vi "GLIMPSE Sequence Save.vi"(5 "Go? (F)":bool, 6 "Header file data":T2 {"Pixel depth" items=["8 bits", "16 bits", "Float", "Complex", "RGB", "HSL"]; "time of 1st frame, \nsec since 1/1/04" format="%.2f"}, 8 "Acquisition refnum array":refnum<file>[](array[refnum]), 9 "Black/White Levels":cluster{ext, ext}(slide)={1.0, 65535.0} scale=1.0..65535.0) -> ()   [LabVIEW 2015]
doc: "Saves a sequence either as a single movied file (SEQ, Stacked TIFF, or AVI) or as a directory full of individual frame images (Multiple TIFF). If more than one AOI is specified, each is saved in a separate, sequentially numbered file or directory. For stacked TIFF or AVI formats, also saves a separate .mat file with time information etc. See Save sequence file into movie.vi for information on the file format."
uses:
  Header file data.ctl
  Seq file v 1/Offset table.ctl
  Seq file v 1/Offset.ctl
  Seq file v 1/file number.ctl
  Header2 file data.ctl
  GLIMPSE Globals.vi
  AOI/AOI List Globals.vi
panel:
  out "Header2 file data 2":T1
  in  "Header2 file data":T1
  in  "AVI AOI Overlay\n(\"Entire Frames\" only)":bool
  in  "AVI Frames Per Second":u32=30
  out "Keep acquisition files open at end":bool=TRUE
  in  "Change File":bool
  out "Current movie directory":path=path "d:/1.glimpse"
  in  "AOI Options":i32(listbox)=1
  in  "stop":bool
  in  "Description Info (SEQ and stacked TIFF formats)":string
  in  "To":u32
  in  "From":u32
  in  "Frame Range Options":i32(listbox)
  in  "File Format Options":i32(listbox)
  # "Make any changes required, then press"
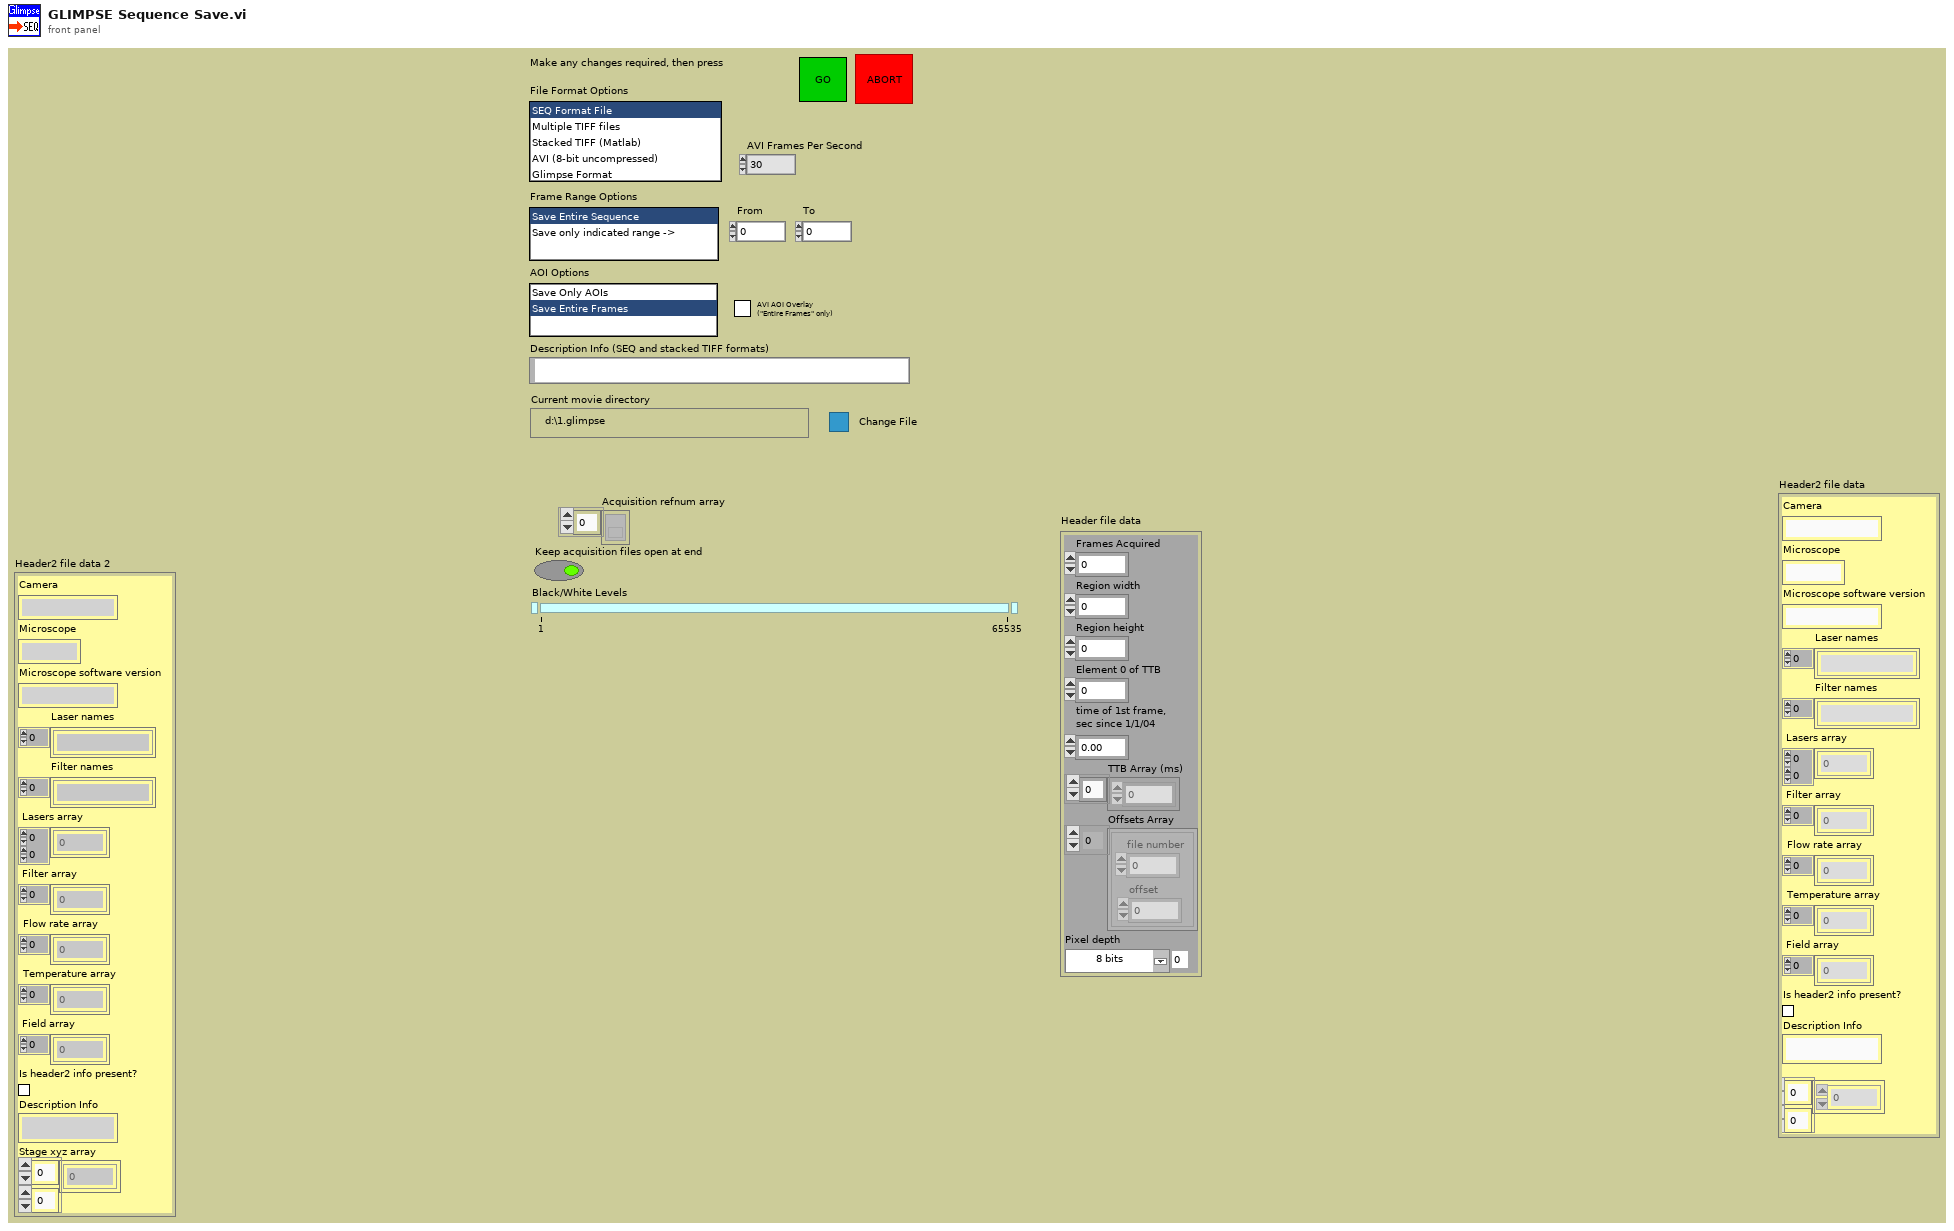
[diagram p1: front panel]
types:
  T1 = typedef "Header2 file data.ctl" = cluster{"Camera":string, "Microscope":string, "Microscope software version":string, "Laser names":string[], "Filter names":string[], "Lasers array":u16[][], "Filter array":u16[], "Flow rate array":dbl[], "Temperature array":dbl[], "Field array":u16[], "Is header2 info present?":bool, "Description Info":string, "Stage xyz array":dbl[][]}
  T2 = typedef "Header file data.ctl" = cluster{"Frames Acquired":u32, "Region width":i32, "Region height":i32, "Element 0 of TTB":u32, "time of 1st frame, \nsec since 1/1/04":dbl, "TTB Array (ms)":u32[], "Offsets Array":T3, "Pixel depth":u32}
  T3 = typedef "Offset table.ctl" = cluster{"offset":T4, "file number":T5}[]
  T4 = typedef "Offset.ctl" = i32
  T5 = typedef "file number.ctl" = u8
  T6 = enum16{"Frames", "Fields, Odd 1st", "Fields, Even 1st", "Fields, Averaged"}
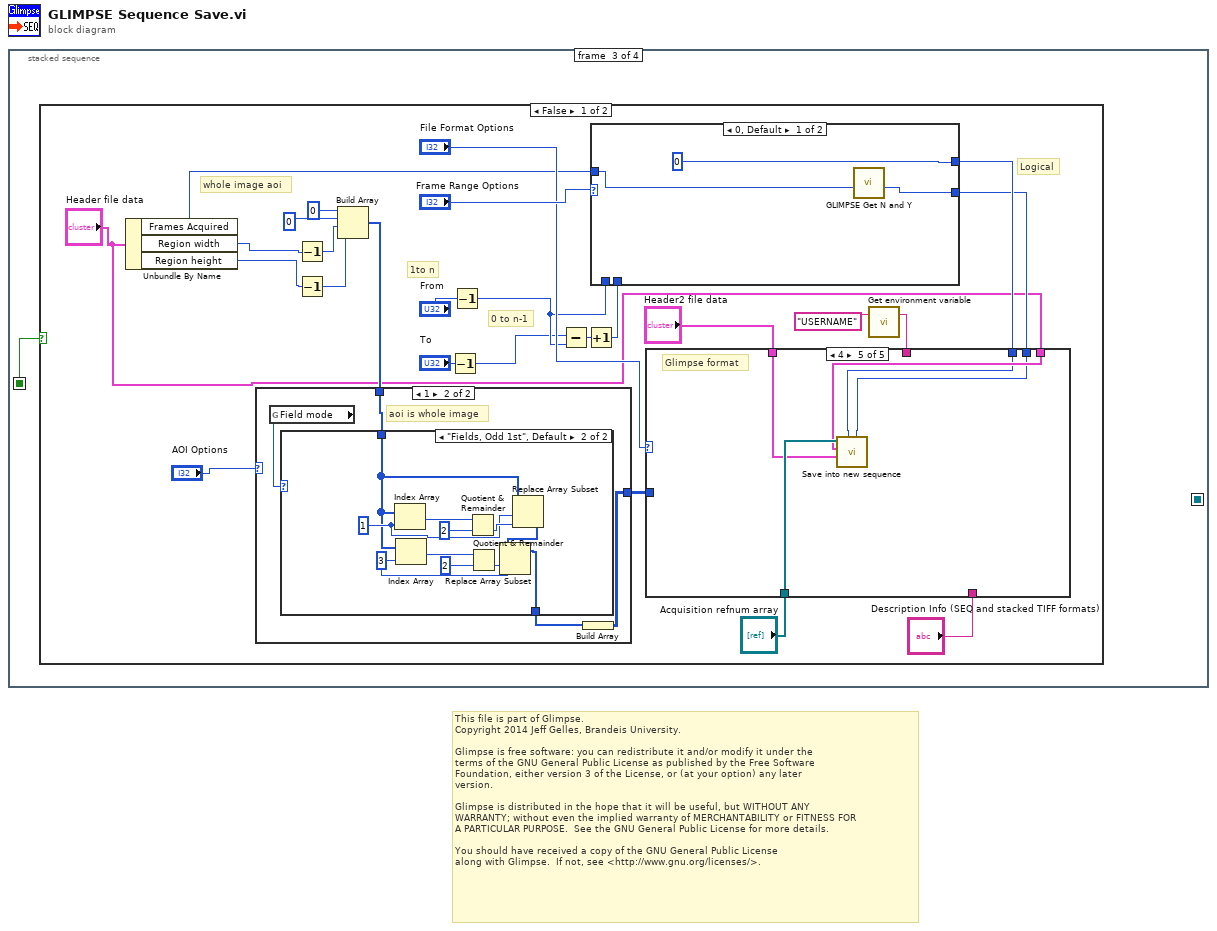
[diagram p0: block diagram]
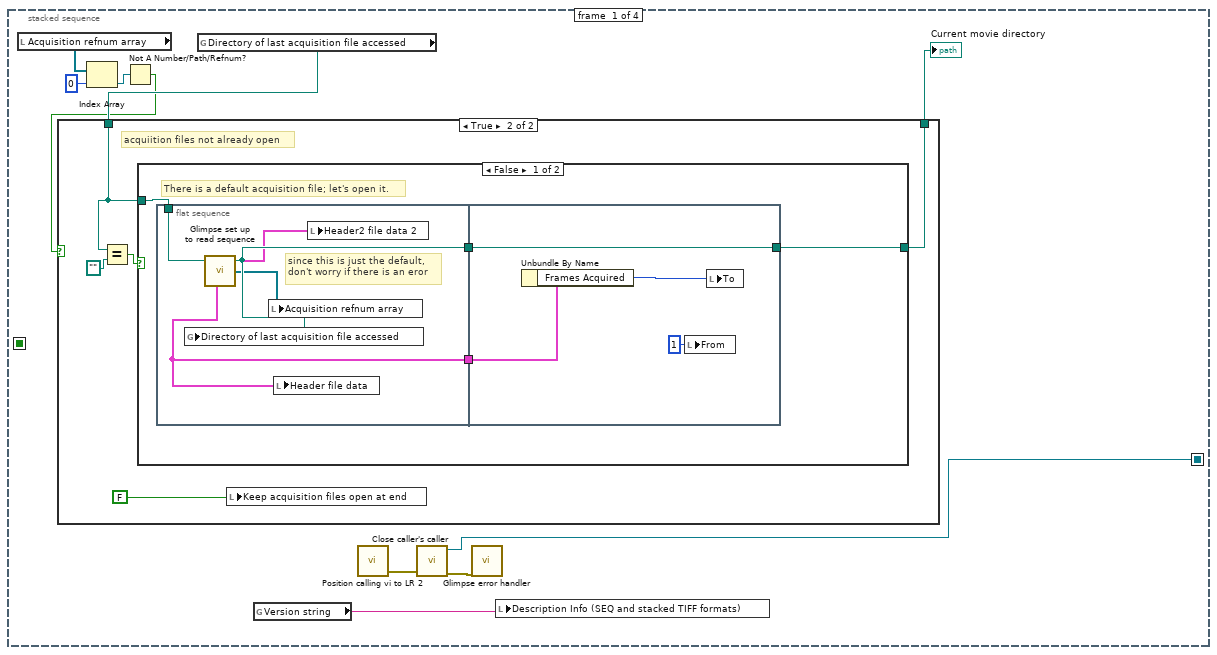
[diagram p2: hidden frame]
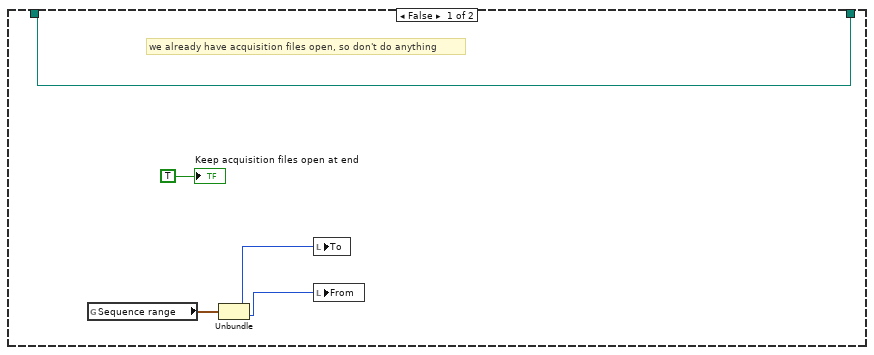
[diagram p3: hidden frame]
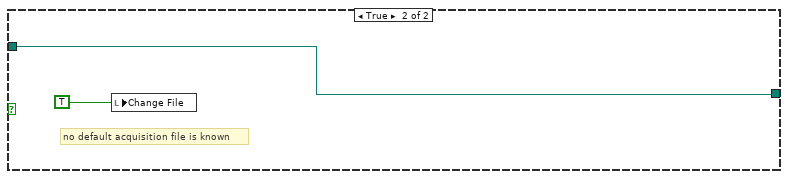
[diagram p4: hidden frame]
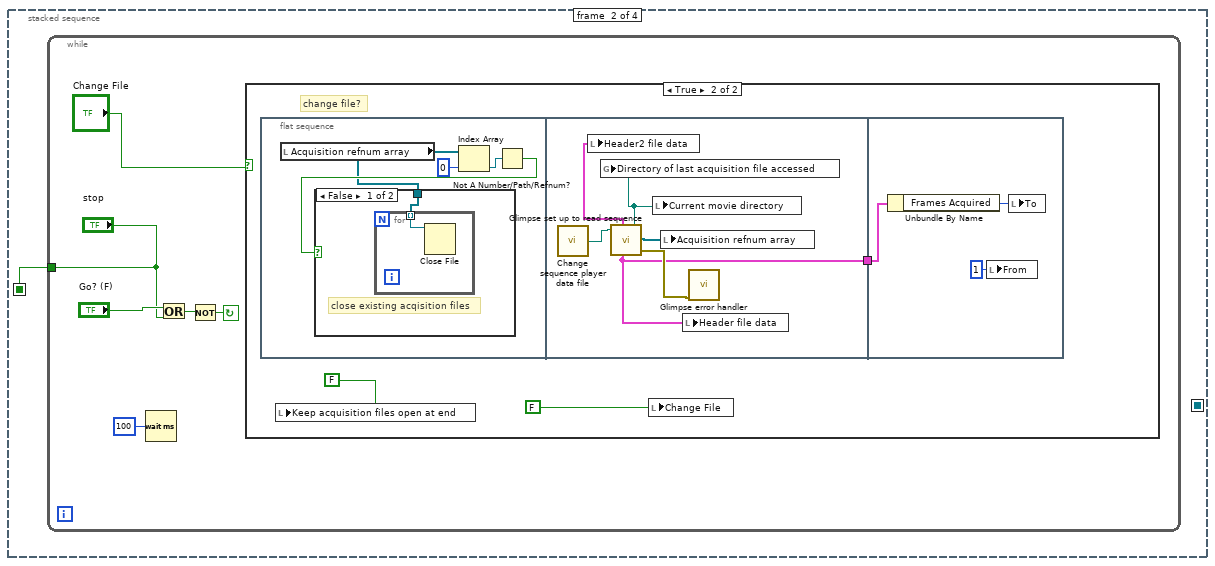
[diagram p5: hidden frame]
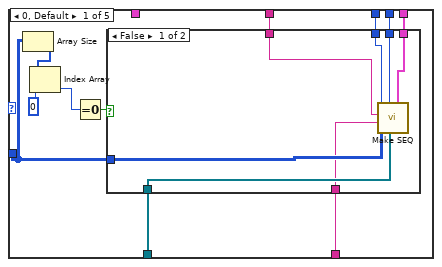
[diagram p8: hidden frame]
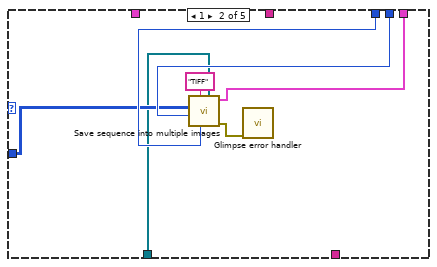
[diagram p10: hidden frame]
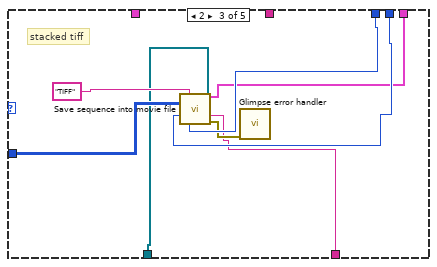
[diagram p11: hidden frame]
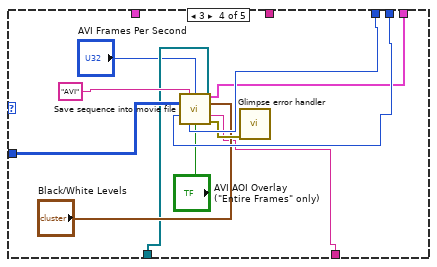
[diagram p12: hidden frame]
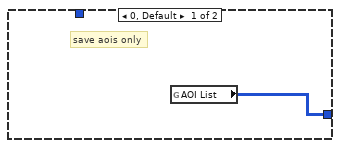
[diagram p13: hidden frame]
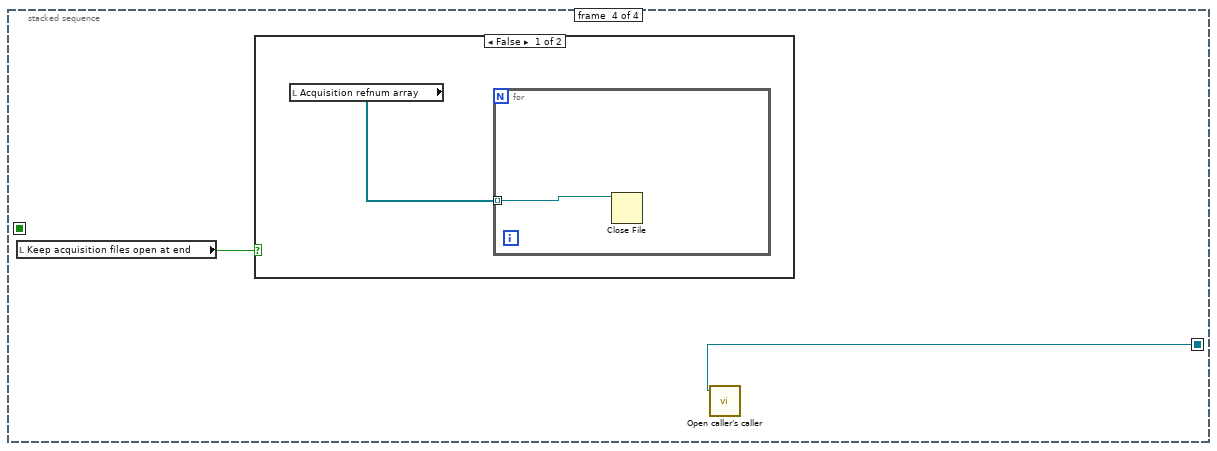
[diagram p17: hidden frame]
diagram:
  # "This file is part of Glimpse. \nCopyright 2014 Jeff Gelles, Brandeis University.    \n\nGlimpse is free software: you can redistribute it and/or modify it under the \nterms of the GNU General Public License as published by the Free Software \nFoundation, either version 3 of the License, or (at your option) any later \nversion.\n\nGlimpse is distributed in the hope that it will be useful, but WITHOUT ANY \nWARRANTY; without even the implied warranty of MERCHANTABILITY or FITNESS FOR \nA PARTICULAR PURPOSE.  See the GNU General Public License for more details.\n\nYou should have received a copy of the GNU General Public License\nalong with Glimpse.  If not, see <http://www.gnu.org/licenses/>."
  n1 = stacked-sequence {
    seq-local: [_ w36 _ _] -> [_ _ w61 _]
    seq-local: [w1 _ _ _] -> [_ _ _ w159]
    frame #0 {
      n2 = local read "Acquisition refnum array"() -> (w8:refnum<file>[])
      n3 = Index Array(array=w8, index=0) -> (element=w6:refnum<file>)
      n4 = Not A Number/Path/Refnum?(number/path/refnum=w6) -> (NaN/Path/Refnum?=w5:bool)
      n5 = global read "GLIMPSE Globals.vi" "Directory of last acquisition file accessed"() -> (w10:path)
      n6 = case shown="True" w5 {
        tunnel: w10 -> [w15 w18]
        tunnel: [w15 w17] -> w9
        frame False {
          # "we already have acquisition files open, so don't do anything"
          n7 = global read "GLIMPSE Globals.vi" "Sequence range"() -> (w13:cluster{i16, i16})
          n8 = Unbundle(w13) -> (w12:i16, w11:i16)
          n9 = local write "To"(w12) -> ()
          n10 = local write "From"(w11) -> ()
          "Keep acquisition files open at end" <- TRUE
        }
        frame True {
          # "acquiition files not already open"
          n11 = Equal?(x=w18, y=path "") -> (x = y?=w19:bool)
          n12 = case shown="False" w19 {
            tunnel: w18 -> [w24 w34]
            tunnel: [w23 w34] -> w17
            frame False {
              # "There is a default acquisition file; let's open it."
              n13 = flat-sequence {
                tunnel: w24 -> [w29]
                tunnel: [w28] -> w22
                tunnel: [w26] -> w21
                tunnel: [w32] -> w23
                tunnel: w22 -> [w32]
                tunnel: w21 -> [w31]
                frame #0 {
                  # "since this is just the default,\ndon't worry if there is an eror"
                  n14 = call "Glimpse set up to read sequence.vi"("acquisition directory path"=w29) -> ("Header2 file data out"=w25:T1, "Header file data out"=w26:T2, "acquisition directory path out"=w28:path, "Acquisition refnum array"=w27:refnum<file>[])  [unwired: 1 in, 2 out]
                  n15 = global write "GLIMPSE Globals.vi" "Directory of last acquisition file accessed"(w28) -> ()
                  n16 = local write "Acquisition refnum array"(w27) -> ()
                  n17 = local write "Header file data"(w26) -> ()
                  n18 = local write "Header2 file data 2"(w25) -> ()
                }
                frame #1 {
                  n19 = Unbundle By Name(w31) -> ("Frames Acquired"=w30:u32)
                  n20 = local write "From"(u16 1 ("From")) -> ()
                  n21 = local write "To"(w30) -> ()
                }
              }
            }
            frame True {
              # "no default acquisition file is known"
              n22 = local write "Change File"(TRUE) -> ()
            }
          }
          n23 = local write "Keep acquisition files open at end"(FALSE) -> ()
        }
      }
      "Current movie directory" <- w9
      n24 = global read "GLIMPSE Globals.vi" "Version string"() -> (w4:string)
      n25 = call "Position calling vi to LR 2.vi"() -> ("error out"=w3:errorcluster)  [unwired: 2 in, 3 out]
      n26 = call "Close caller's caller.vi"("error in (no error)"=w3) -> ("error out"=w2:errorcluster, "vi reference"=w1:refnum<vi>)  [unwired: 6 out]
      n27 = call "Glimpse error handler.vi"("error in"=w2) -> ()  [unwired: 1 in, 6 out]
      n28 = local write "Description Info (SEQ and stacked TIFF formats)"(w4) -> ()
    }
    frame #1 {
      n29 = while {
        tunnel: ["stop"] -> w36
        stop <- w41 continue-if-true
        n30 = Wait (ms)(milliseconds to wait=u32 100) -> ()  [unwired: 1 out]
        n31 = Or(x="Go? (F)", y="stop") -> (x .or. y?=w39:bool)
        n32 = Not(x=w39) -> (.not. x?=w41:bool)
        n33 = case shown="True" "Change File" {
          frame False {
          }
          frame True {
            # "change file?"
            n34 = flat-sequence {
              tunnel: [w53] -> w43
              tunnel: w43 -> [w59]
              frame #0 {
                n35 = local read "Acquisition refnum array"() -> (w46:refnum<file>[])
                n36 = Index Array(array=w46, index=0) -> (element=w48:refnum<file>)
                n37 = Not A Number/Path/Refnum?(number/path/refnum=w48) -> (NaN/Path/Refnum?=w47:bool)
                n38 = case shown="False" w47 {
                  tunnel: w46 -> [w50 _]
                  frame False {
                    # "close existing acqisition files"
                    n39 = for {
                      tunnel: w50 -> [w51] mode=indexing
                      n40 = Close File(refnum=w51) -> ()  [unwired: 1 in, 2 out]
                    }
                  }
                  frame True {
                  }
                }
              }
              frame #1 {
                n41 = call "Change sequence player data file.vi"() -> ("File path out"=w57:path)  [unwired: 1 in, 4 out]
                n42 = call "Glimpse set up to read sequence.vi"("acquisition directory path"=w57) -> ("Header2 file data out"=w52:T1, "Header file data out"=w53:T2, "acquisition directory path out"=w56:path, "Acquisition refnum array"=w55:refnum<file>[], "error out"=w54:errorcluster)  [unwired: 1 in, 1 out]
                n43 = local write "Header2 file data"(w52) -> ()
                n44 = global write "GLIMPSE Globals.vi" "Directory of last acquisition file accessed"(w56) -> ()
                n45 = local write "Current movie directory"(w56) -> ()
                n46 = local write "Acquisition refnum array"(w55) -> ()
                n47 = local write "Header file data"(w53) -> ()
                n48 = call "Glimpse error handler.vi"("error in"=w54) -> ()  [unwired: 1 in, 6 out]
              }
              frame #2 {
                n49 = Unbundle By Name(w59) -> ("Frames Acquired"=w58:u32)
                n50 = local write "From"(u16 1 ("From")) -> ()
                n51 = local write "To"(w58) -> ()
              }
            }
            n52 = local write "Keep acquisition files open at end"(FALSE) -> ()
            n53 = local write "Change File"(FALSE) -> ()
          }
        }
      }
    }
    frame #2 {
      n54 = case shown="False" w61 {
        frame False {
          # "0 to n-1"
          # "1to n"
          # "whole image aoi"
          # "Logical"
          n55 = Unbundle By Name("Header file data") -> ("Frames Acquired"=w68:u32, "Region width"=w70:i32, "Region height"=w69:i32)
          n56 = Decrement(x=w70) -> (x-1=w74:i32)
          n57 = Decrement(x=w69) -> (x-1=w72:i32)
          n58 = Build Array(u16 0 ("element"), u16 0 ("element"), w74, w72) -> (w71:i32[])
          n59 = case shown="1" "AOI Options" {
            tunnel: [w137 w141] -> w82
            tunnel: w71 -> [_ w138]
            frame 0, Default {
              # "save aois only"
              n60 = global read "AOI List Globals.vi" "AOI List"() -> (w137:u16[][])
            }
            frame 1 {
              # "aoi is whole image"
              n61 = global read "GLIMPSE Globals.vi" "Field mode"() -> (w140:T6)
              n62 = case shown="\"Fields, Odd 1st\", Default" w140 {
                tunnel: [w142 w146] -> w139
                tunnel: w138 -> [w142 w143]
                frame "Frames" {
                }
                frame "Fields, Odd 1st", Default {
                  w151 = 3 ("Index")
                  w147 = 1 ("Index")
                  n63 = Index Array(array=w143, index=w147) -> (element=w145:i32)
                  n64 = Index Array(array=w143, index=w151) -> (element=w144:i32)
                  n65 = Quotient & Remainder(x=w145, y=i8 2) -> (floor(x/y)=w152:i32)  [unwired: 1 out]
                  n66 = Quotient & Remainder(x=w144, y=i8 2) -> (floor(x/y)=w148:i32)  [unwired: 1 out]
                  n67 = Replace Array Subset(array=w143, new element=w152, index=w147) -> (w149:i32[])
                  n68 = Replace Array Subset(array=w149, new element=w148, index=w151) -> (w146:i32[])
                }
              }
              n69 = Build Array(w139) -> (w141:i32[][])
            }
          }
          n70 = Decrement(x="To") -> (x-1=w78:u32)
          n71 = Decrement(x="From") -> (x-1=w79:u32)
          n72 = Subtract(x=w78, y=w79) -> (x-y=w86:u32)
          n73 = Increment(x=w86) -> (x+1=w85:u32)
          n74 = case shown="0, Default" "Frame Range Options" {
            tunnel: w79 -> [_ w158]
            tunnel: w85 -> [_ w157]
            tunnel: [u32 0 w158] -> w77
            tunnel: [w155 w157] -> w76
            tunnel: w68 -> [w154 _]
            frame 0, Default {
              n75 = call "GLIMPSE Get N and Y.vi"("# of Frames In (Phys)"=w154) -> ("# of Frames Out (Log)"=w155:u32)  [unwired: 2 in, 4 out]
            }
            frame 1 {
            }
          }
          n76 = call "Get environment variable.vi"("Variable name"="USERNAME") -> ("Value"=w63:string)  [unwired: 2 out]
          n77 = case shown="4" "File Format Options" {
            tunnel: w82 -> [w98 w108 w120 w131 _]
            tunnel: w76 -> [w93 w110 w116 w127 w132]
            tunnel: w77 -> [w92 w111 w119 w130 w133]
            tunnel: "Header file data" -> [w91 w107 w115 w126 w134]
            tunnel: "Acquisition refnum array" -> [w90 w106 w114 w124 w136]
            tunnel: "Description Info (SEQ and stacked TIFF formats)" -> [w89 _ w113 w123 _]
            tunnel: w63 -> [w88 _ _ _ _]
            tunnel: "Header2 file data" -> [_ _ _ _ w135]
            frame 0, Default {
              n78 = Array Size(array=w98) -> (size(s)=w97:i32[])
              n79 = Index Array(array=w97, index=0) -> (element=w95:i32)
              n80 = Equal To 0?(x=w95) -> (x = 0?=w94:bool)
              n81 = case shown="False" w94 {
                tunnel: w98 -> [w105 _]
                tunnel: w93 -> [w103 _]
                tunnel: w92 -> [w104 _]
                tunnel: w91 -> [w102 _]
                tunnel: w90 -> [w101 _]
                tunnel: w89 -> [w100 _]
                tunnel: w88 -> [w99 _]
                frame False {
                  n82 = call "Make SEQ.vi"("Header file data"=w102, "Acqisition files refnums"=w101, "Number of images"=w103, "AOI List"=w105, "Description"=w100, "User Info"=w99, "First image number (start 0)"=w104) -> ()  [unwired: 1 in, 3 out]
                }
                frame True {
                }
              }
            }
            frame 1 {
              n83 = call "Save sequence into multiple images.vi"("Header file data"=w107, "Acqisition files refnums"=w106, "starting frame number to save"=w111, "File Format"="TIFF" ("File Type"), "Number of frames to save"=w110, "AOI List"=w108) -> ("error out"=w109:errorcluster)  [unwired: 2 in, 2 out]
              n84 = call "Glimpse error handler.vi"("error in"=w109) -> ()  [unwired: 1 in, 6 out]
            }
            frame 2 {
              # "stacked tiff"
              n85 = call "Save sequence into movie file.vi"("File Format"="TIFF" ("File Type"), "Header file data"=w115, "AOI List"=w120, "Acqisition files refnums"=w114, "Number of frames to save"=w116, "Description Info (SEQ and stacked TIFF formats)"=w113, "starting frame number to save"=w119) -> ("error out"=w118:errorcluster)  [unwired: 5 in, 3 out]
              n86 = call "Glimpse error handler.vi"("error in"=w118) -> ()  [unwired: 1 in, 6 out]
            }
            frame 3 {
              n87 = call "Save sequence into movie file.vi"("File Format"="AVI" ("File Type"), "AVI Frames Per Second"="AVI Frames Per Second", "Header file data"=w126, "AOI List"=w131, "Black/White Levels"="Black/White Levels", "Acqisition files refnums"=w124, "Number of frames to save"=w127, "Description Info (SEQ and stacked TIFF formats)"=w123, "starting frame number to save"=w130, "AOI Overlay?"="AVI AOI Overlay\n(\"Entire Frames\" only)") -> ("error out"=w129:errorcluster)  [unwired: 2 in, 3 out]
              n88 = call "Glimpse error handler.vi"("error in"=w129) -> ()  [unwired: 1 in, 6 out]
            }
            frame 4 {
              # "Glimpse format"
              n89 = call "Save into new sequence.vi"("number of images to save"=w132, "First image to save (start with 0)"=w133, "Header2 file data"=w135, "Header file data"=w134, "Acquisition refnum array"=w136) -> ()  [unwired: 7 in]
            }
          }
        }
        frame True {
        }
      }
    }
    frame #3 {
      n90 = local read "Keep acquisition files open at end"() -> (w160:bool)
      n91 = case shown="False" w160 {
        frame False {
          n92 = local read "Acquisition refnum array"() -> (w161:refnum<file>[])
          n93 = for {
            tunnel: w161 -> [w162] mode=indexing
            n94 = Close File(refnum=w162) -> ()  [unwired: 1 in, 2 out]
          }
        }
        frame True {
        }
      }
      n95 = call "Open caller's caller.vi"("vi reference"=w159) -> ()  [unwired: 1 in, 7 out]
    }
  }
